vi "Shooter_Operator_Assist.vi"(0 "Turret Aimed":bool, 5 "Ball In Position":bool, 7 "Shooter Motor Speed Good":bool, 9 "Shoot Command":bool, 11 "Start":bool) -> (4 "BottomFeeder":bool=TRUE, 6 "ShooterMotor":bool=TRUE, 8 "TurretMotor":bool=TRUE, 10 "TopFeeder":bool=TRUE)   [LabVIEW 2016]
uses:
  TypeDefs/ShooterState_Type.ctl
panel:
  in  "ManualOverride":bool=TRUE
  out "ShooterState":T1
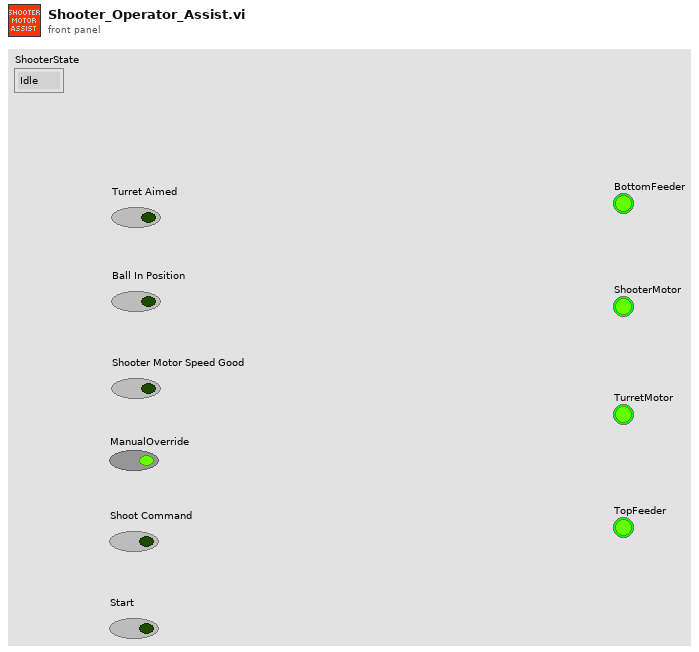
[diagram p1: front panel]
types:
  T1 = typedef "ShooterState_Type.ctl" = enum16{"Idle", "Recover", "Shoot", "QueueFuel"}
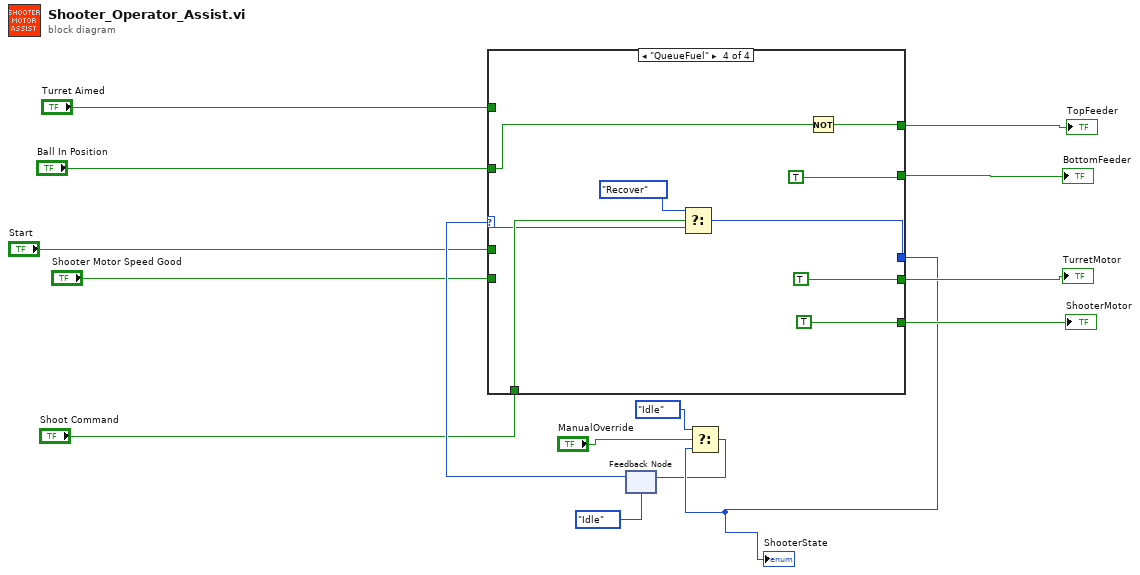
[diagram p0: block diagram]
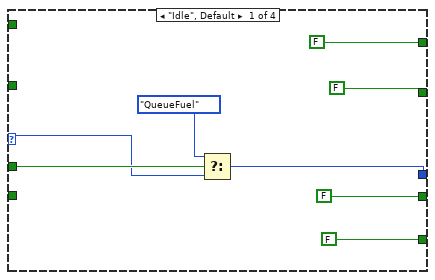
[diagram p2: hidden frame]
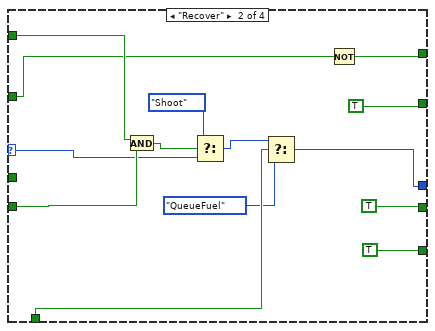
[diagram p3: hidden frame]
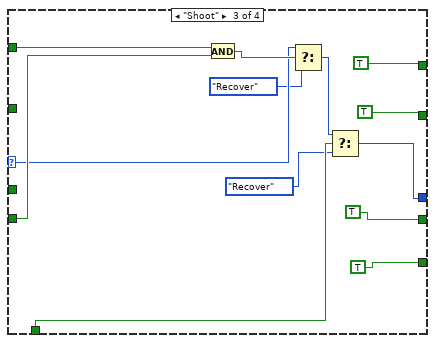
[diagram p4: hidden frame]
diagram:
  n1 = feedback #1(ShooterState_Type."Idle" ("t")) -> (w15:T1)
  n2 = case shown="\"QueueFuel\"" w15 {
    selector: w15 -> [w22 w34 w47 w58]
    tunnel: [w21 w31 w42 w56] -> w4
    tunnel: "Start" -> [w23 _ _ _]
    tunnel: "Shoot Command" -> [_ w30 w45 w59]
    tunnel: "Shooter Motor Speed Good" -> [_ w37 w48 _]
    tunnel: "Turret Aimed" -> [_ w36 w50 _]
    tunnel: "Ball In Position" -> [_ w28 _ w51]
    tunnel: [FALSE w27 TRUE w52] -> w9
    tunnel: [FALSE TRUE TRUE TRUE] -> w8
    tunnel: [FALSE TRUE TRUE TRUE] -> w7
    tunnel: [FALSE TRUE TRUE TRUE] -> w6
    frame "Idle", Default {
      n3 = Select(t=ShooterState_Type."QueueFuel", s=w23, f=w22) -> (s? t:f=w21:T1)
    }
    frame "Recover" {
      n4 = And(x=w36, y=w37) -> (x .and. y?=w35:bool)
      n5 = Select(t=ShooterState_Type."Shoot", s=w35, f=w34) -> (s? t:f=w32:T1)
      n6 = Select(t=w32, s=w30, f=ShooterState_Type."QueueFuel") -> (s? t:f=w31:T1)
      n7 = Not(x=w28) -> (.not. x?=w27:bool)
    }
    frame "Shoot" {
      n8 = And(x=w50, y=w48) -> (x .and. y?=w49:bool)
      n9 = Select(t=w47, s=w49, f=ShooterState_Type."Recover") -> (s? t:f=w44:T1)
      n10 = Select(t=w44, s=w45, f=ShooterState_Type."Recover") -> (s? t:f=w42:T1)
    }
    frame "QueueFuel" {
      n11 = Select(t=ShooterState_Type."Recover", s=w59, f=w58) -> (s? t:f=w56:T1)
      n12 = Not(x=w51) -> (.not. x?=w52:bool)
    }
  }
  "ShooterState" <- w4
  "TopFeeder" <- w9
  "BottomFeeder" <- w8
  "TurretMotor" <- w7
  "ShooterMotor" <- w6
  n13 = Select(t=ShooterState_Type."Idle", s="ManualOverride", f=w4) -> (s? t:f=w3:T1)
  n14 = feedback-in #1(w3) -> ()
